vi "FlatToRichauth_ValidateTokenRequest.vi"(5 "OutputClusterType":T1, 11 "InputCluster":T2) -> (3 "OutputCluster":T1)   [LabVIEW 2020, in "grpc-auth_client.lvlib"]
uses:
  auth_ValidateTokenRequest_Flat.ctl
  auth_ValidateTokenRequest.ctl
  grpc-auth_client.lvlib
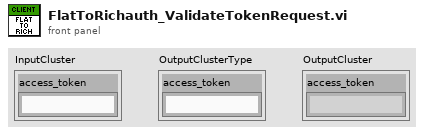
[diagram p1: front panel]
types:
  T1 = typedef "grpc-auth_client.lvlib/auth_ValidateTokenRequest.ctl" = cluster{"access_token":string}
  T2 = typedef "grpc-auth_client.lvlib/auth_ValidateTokenRequest_Flat.ctl" = cluster{"access_token":string}
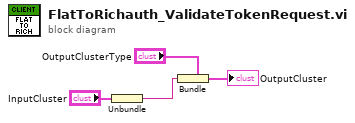
[diagram p0: block diagram]
diagram:
  n1 = Unbundle "Unbundle"("InputCluster") -> ("access_token"=w1:string)
  n2 = Bundle "Bundle"(cluster="OutputClusterType", "access_token"=w1) -> (→"OutputCluster":T1)
